vi "Update Button Images.vi"(4 "New Index":i32=-1, 6 "Old Index":i32=-1, 7 "Force Regen":bool, 8 "error in (no error)":errorcluster, 9 "Old State":T1={"Buttons Displayed"=0, "Button States"=[], "Button Size"=0, "Button Style"=enum."Classic", "Active Button"=0, "Force Regen?"=FALSE, "Tip String Ref"=refnum} caption="State", 10 "New State":T1={"Buttons Displayed"=0, "Button States"=[], "Button Size"=0, "Button Style"=enum."Classic", "Active Button"=0, "Force Regen?"=FALSE, "Tip String Ref"=refnum} caption="State", 11 "Images In":picture[](array[picture])) -> (0 "error out":errorcluster, 2 "State Out":T1={"Buttons Displayed"=0, "Button States"=[], "Button Size"=0, "Button Style"=enum."Classic", "Active Button"=0, "Force Regen?"=FALSE, "Tip String Ref"=refnum} caption="State", 3 "Images Out":picture[](array[picture]))   [LabVIEW 2012, in "Toolbar.xctl"]
doc: "Works out a new button image, either completely regenerating the image from the drawing data or if it can, just by switching between the pre-cached images for each state."
uses:
  Toolbar.xctl
  Toolbar State.ctl
  Button_Class/Button.lvclass
  Button_Class/Type Defs/Button Style.ctl
  <vilib>/Analysis/1siggen.llb/Ramp Pattern by Samples.vi
  <vilib>/Analysis/NI_AALBase.lvlib
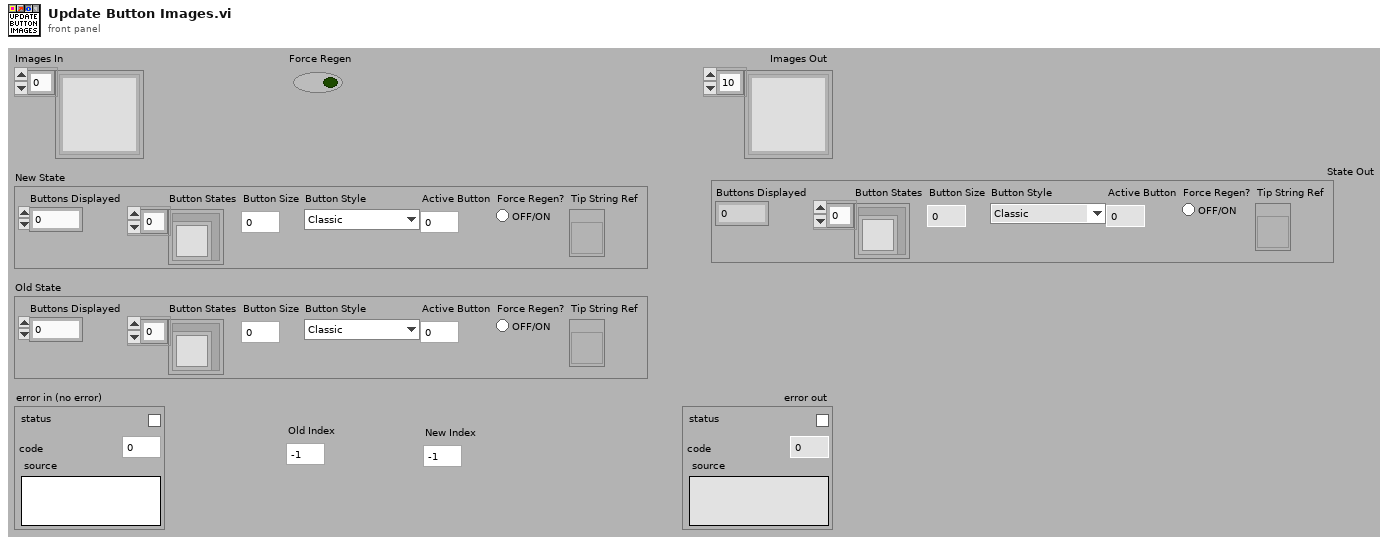
[diagram p1: front panel]
types:
  T1 = typedef "Toolbar.xctl/Toolbar State.ctl" = cluster{"Buttons Displayed":i32, "Button States":refnum<class "Button.lvclass">[], "Button Size":i32, "Button Style":T2, "Active Button":i32, "Force Regen?":bool, "Tip String Ref":refnum<vi>}
  T2 = typedef "Button.lvclass/Button Style.ctl" = enum16{"System", "Modern", "Classic", "Rounded", "Silver", "Ni Theme", "Metallic"}
  T3 = typedef "Button.lvclass/Button Status.ctl" = enum16{"Off", "Hover", "On", "Disabled"}
  T4 = typedef "Button.lvclass/Button Type.ctl" = enum16{"Transitory", "Latching"}
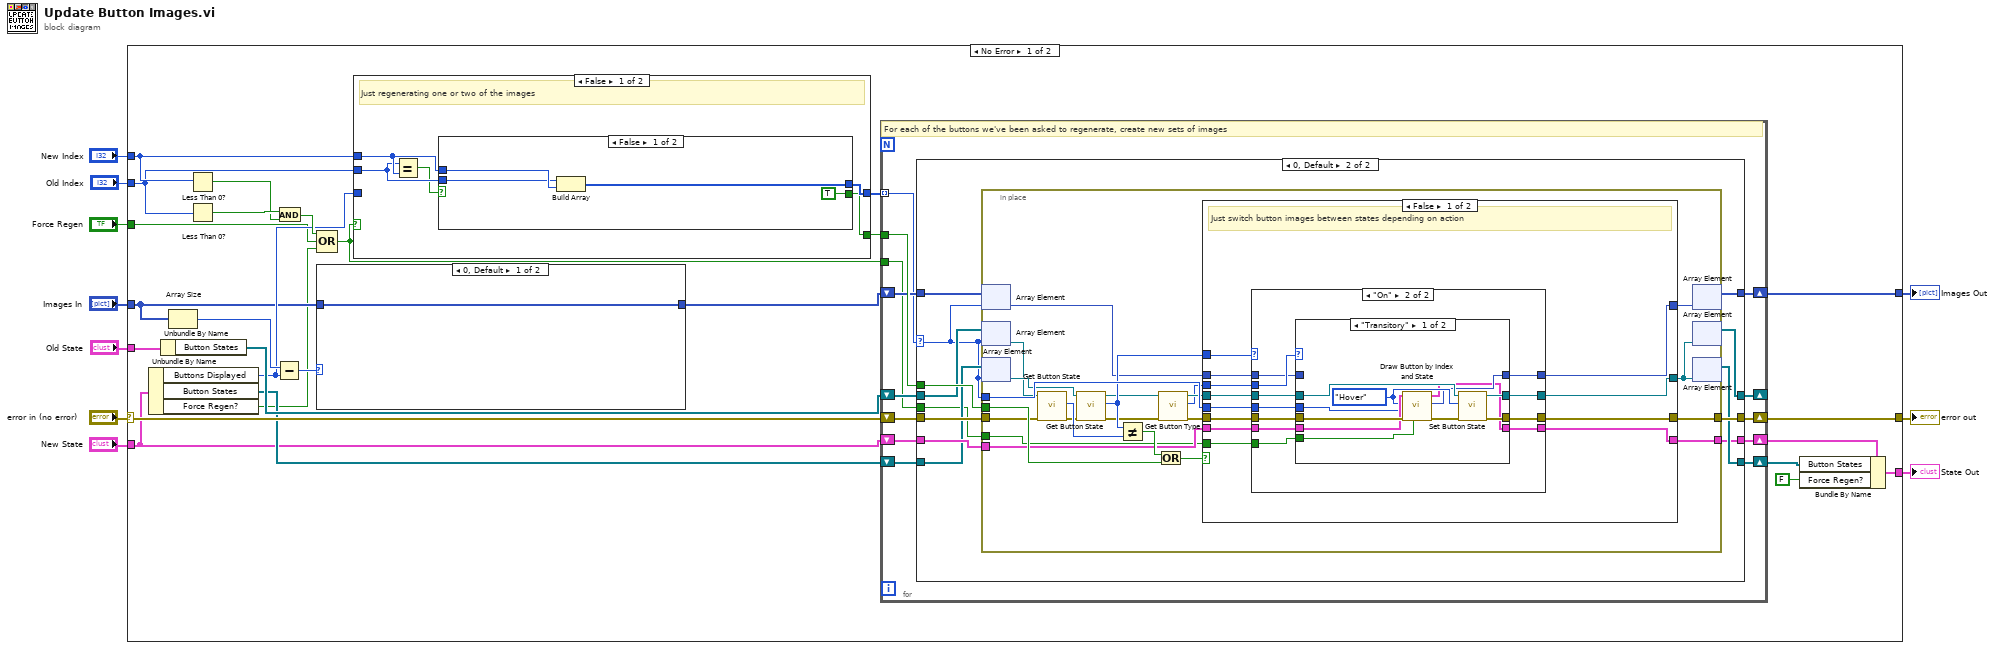
[diagram p0: block diagram]
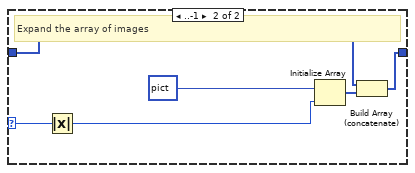
[diagram p2: hidden frame]
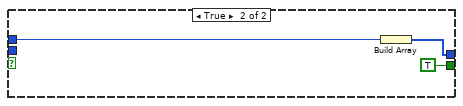
[diagram p3: hidden frame]
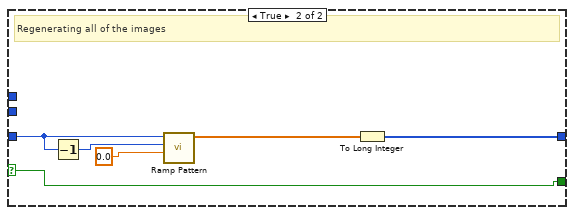
[diagram p4: hidden frame]
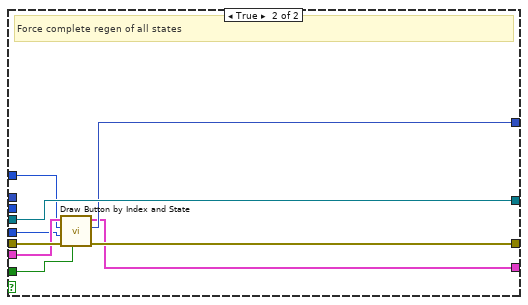
[diagram p8: hidden frame]
diagram:
  n1 = case shown="No Error" "error in (no error)" {
    selector: "error in (no error)" -> [w34 w167]
    tunnel: "New State" -> [w17 w166]
    tunnel: [w33 w167] -> w9
    tunnel: "Old State" -> [w36 _]
    tunnel: "Images In" -> [w19 _]
    tunnel: [w35 _] -> w7
    tunnel: [w32 w166] -> w6
    tunnel: "Force Regen" -> [w13 _]
    tunnel: "New Index" -> [w15 _]
    tunnel: "Old Index" -> [w14 _]
    frame No Error {
      n2 = Unbundle By Name(w17) -> ("Buttons Displayed"=w21:i32, "Button States"=w29:refnum<class "Button.lvclass">[], "Force Regen?"=w12:bool)
      n3 = Unbundle By Name(w36) -> ("Button States"=w30:refnum<class "Button.lvclass">[])
      n4 = Array Size(array=w19) -> (size(s)=w22:i32)
      n5 = Less Than 0?(x=w15) -> (x < 0?=w26:bool)
      n6 = Less Than 0?(x=w14) -> (x < 0?=w27:bool)
      n7 = Subtract(x=w22, y=w21) -> (x-y=w20:i32)
      n8 = And(x=w27, y=w26) -> (x .and. y?=w25:bool)
      n9 = Compound Arithmetic op=OR(w25, w13, w12) -> (w11:bool)
      n10 = case shown="0, Default" w20 {
        selector: w20 -> [_ w42]
        tunnel: w19 -> [w37 w39]
        tunnel: [w37 w38] -> w18
        frame 0, Default {
        }
        frame ..-1 {
          # "Expand the array of images"
          n11 = Absolute Value(x=w42) -> (abs(x)=w43:i32)
          n12 = Initialize Array(picture data[5B] ("On Picture"), w43) -> (w40:picture[])
          n13 = Build Array (concatenate)(w39, w40) -> (w38:picture[])
        }
      }
      n14 = case shown="False" w11 {
        selector: w11 -> [_ w56]
        tunnel: w21 -> [_ w60]
        tunnel: [w48 w57] -> w28
        tunnel: w14 -> [w45 _]
        tunnel: w15 -> [w46 _]
        tunnel: [w47 w56] -> w24
        frame False {
          # "Just regenerating one or two of the images"
          n15 = Equal?(x=w45, y=w46) -> (x = y?=w44:bool)
          n16 = case shown="False" w44 {
            tunnel: [w52 w54] -> w48
            tunnel: [TRUE TRUE] -> w47
            tunnel: w46 -> [w50 w55]
            tunnel: w45 -> [w49 _]
            frame False {
              n17 = Build Array(w49, w50) -> (w52:i32[])
            }
            frame True {
              n18 = Build Array(w55) -> (w54:i32[])
            }
          }
        }
        frame True {
          # "Regenerating all of the images"
          n19 = Decrement(x=w60) -> (x-1=w61:i32)
          n20 = call-poly <vilib>:"Ramp Pattern.vi"("start"=0.0, "end"=w61, "samples"=w60) -> ("Ramp Pattern"=w58:dbl[])  [unwired: 7 in, 1 out]
          n21 = To Long Integer(number=w58) -> (32bit integer=w57:i32[])
        }
      }
      n22 = for {
        shift-right: [w67] -> w35
        shift-left: w18 -> [w68]
        shift-right: [w74] -> w33
        shift-left: w34 -> [w71]
        tunnel: w24 -> [w73]
        shift-right: [w69] -> w31
        shift-left: w29 -> [w70]
        tunnel: w28 -> [w64] mode=indexing
        shift-right: [w65] -> _
        shift-left: w30 -> [w66]
        shift-right: [w63] -> w16
        shift-left: w17 -> [w72]
        tunnel: w11 -> [w62]
        # "For each of the buttons we've been asked to regenerate, create new sets of images"
        n23 = case shown="0, Default" w64 {
          selector: w64 -> [_ w82]
          tunnel: [w76 w92] -> w74
          tunnel: w73 -> [_ w91]
          tunnel: w72 -> [w75 w90]
          tunnel: w71 -> [w76 w89]
          tunnel: w70 -> [w77 w88]
          tunnel: [w77 w87] -> w69
          tunnel: w68 -> [w78 w86]
          tunnel: [w78 w85] -> w67
          tunnel: w66 -> [w79 w84]
          tunnel: [w79 w83] -> w65
          tunnel: [w75 w81] -> w63
          tunnel: w62 -> [_ w80]
          frame ..-1 {
          }
          frame 0, Default {
            n24 = in-place {
              in-place-border: [w113] -> w92
              in-place-border: w91 -> [w111]
              in-place-border: w90 -> [w110]
              in-place-border: w82 -> [w109]
              in-place-border: w89 -> [w101]
              in-place-border: [w94] -> w81
              in-place-border: w80 -> [w93]
              n25 = in-place-array #1(w86, w82) -> (w98:picture)
              n26 = in-place-array #2(w84, w82) -> (w96:refnum<class "Button.lvclass">)
              n27 = in-place-array #3(w88, w82) -> (w99:refnum<class "Button.lvclass">)
              n28 = call-dynamic "Get Button State.vi"("error in (no error)"=w101, "Button in"=w96) -> ("error out"=w107:errorcluster, "State"=w108:T3)  [unwired: 8 out]
              n29 = call-dynamic "Get Button State.vi"("error in (no error)"=w107, "Button in"=w99) -> ("error out"=w104:errorcluster, "State"=w106:T3, "Button out"=w105:refnum<class "Button.lvclass">)  [unwired: 7 out]
              n30 = Not Equal?(x=w106, y=w108) -> (x != y?=w114:bool)
              n31 = Or(x=w114, y=w111) -> (x .or. y?=w112:bool)
              n32 = call-dynamic "Get Button Type.vi"("error in (no error)"=w104, "Button in"=w105) -> ("error out"=w100:errorcluster, "Type"=w102:T4, "Button out"=w103:refnum<class "Button.lvclass">)  [unwired: 7 out]
              n33 = case shown="False" w112 {
                tunnel: [w121 w163] -> w113
                tunnel: w100 -> [w122 w164]
                tunnel: w106 -> [w126 w161]
                tunnel: w103 -> [w124 w165]
                tunnel: [w123 w165] -> w95
                tunnel: w102 -> [w125 _]
                tunnel: w110 -> [w120 w162]
                tunnel: w109 -> [w119 w160]
                tunnel: w98 -> [w117 _]
                tunnel: [w118 w159] -> w97
                tunnel: [w116 w158] -> w94
                tunnel: w93 -> [w115 w157]
                frame False {
                  # "Just switch button images between states depending on action"
                  n34 = case shown="\"On\"" w126 {
                    tunnel: w124 -> [w130 w139]
                    tunnel: w125 -> [_ w141]
                    tunnel: [w130 w140] -> w123
                    tunnel: w122 -> [w129 w138]
                    tunnel: [w129 w137] -> w121
                    tunnel: w120 -> [w127 w136]
                    tunnel: w119 -> [_ w135]
                    tunnel: [w128 w134] -> w118
                    tunnel: w117 -> [w128 w133]
                    tunnel: [w127 w132] -> w116
                    tunnel: w115 -> [_ w131]
                    frame "Off", Default {
                    }
                    frame "On" {
                      n35 = case shown="\"Transitory\"" w141 {
                        tunnel: [w148 w156] -> w140
                        tunnel: w139 -> [w149 w156]
                        tunnel: w138 -> [w152 w155]
                        tunnel: [w146 w155] -> w137
                        tunnel: w136 -> [w151 w153]
                        tunnel: w135 -> [w145 _]
                        tunnel: [w144 w154] -> w134
                        tunnel: w133 -> [_ w154]
                        tunnel: [w143 w153] -> w132
                        tunnel: w131 -> [w142 _]
                        frame "Transitory" {
                          w150 = enum16{"Off", "Hover", "On", "Disabled"}."Hover" ("State")
                          n36 = call "Draw Button by Index and State.vi"("Force redraw ?"=w142, "error in (no error)"=w152, "index"=w145, "Button State"=w150, "State"=w151) -> ("error out"=w147:errorcluster, "Picture Out"=w144:picture, "State out"=w143:T1)  [unwired: 3 in, 1 out]
                          n37 = call-dynamic "Set Button State.vi"("error in (no error)"=w147, "State"=w150, "Button in"=w149) -> ("error out"=w146:errorcluster, "Button out"=w148:refnum<class "Button.lvclass">)  [unwired: 1 in, 6 out]
                        }
                        frame "Latching", Default {
                        }
                      }
                    }
                  }
                }
                frame True {
                  # "Force complete regen of all states"
                  n38 = call "Draw Button by Index and State.vi"("Force redraw ?"=w157, "error in (no error)"=w164, "index"=w160, "Button State"=w161, "State"=w162) -> ("error out"=w163:errorcluster, "Picture Out"=w159:picture, "State out"=w158:T1)  [unwired: 3 in, 1 out]
                }
              }
              n39 = in-place-array #1(w97) -> (w85:picture[])  [unwired: 1 out]
              n40 = in-place-array #2(w95) -> (w83:refnum<class "Button.lvclass">[])  [unwired: 1 out]
              n41 = in-place-array #3(w95) -> (w87:refnum<class "Button.lvclass">[])  [unwired: 1 out]
            }
          }
        }
      }
      n42 = Bundle By Name(cluster=w16, "Button States"=w31, "Force Regen?"=FALSE) -> (w32:T1)
    }
    frame Error {
    }
  }
  "Images Out" <- w7
  "error out" <- w9
  "State Out" <- w6
